vi "Analog_Read_Ex.vi"() -> ()   [LabVIEW 2026]
panel:
  in  "VISA resource name":refnum<visa-resource-name>
  in  "Stop Button":bool
  in  "Canal Read":u8
  out "Waveform Chart":i32(graph)
  out "error out":errorcluster
  # "Ejemplo: Analog Read"
  # "Descripción: Lee un pin analógico del microcontrolador y muestra el valor en un indicador."
  # "Configuracion"
  # "Indicadores"
  # "Control"
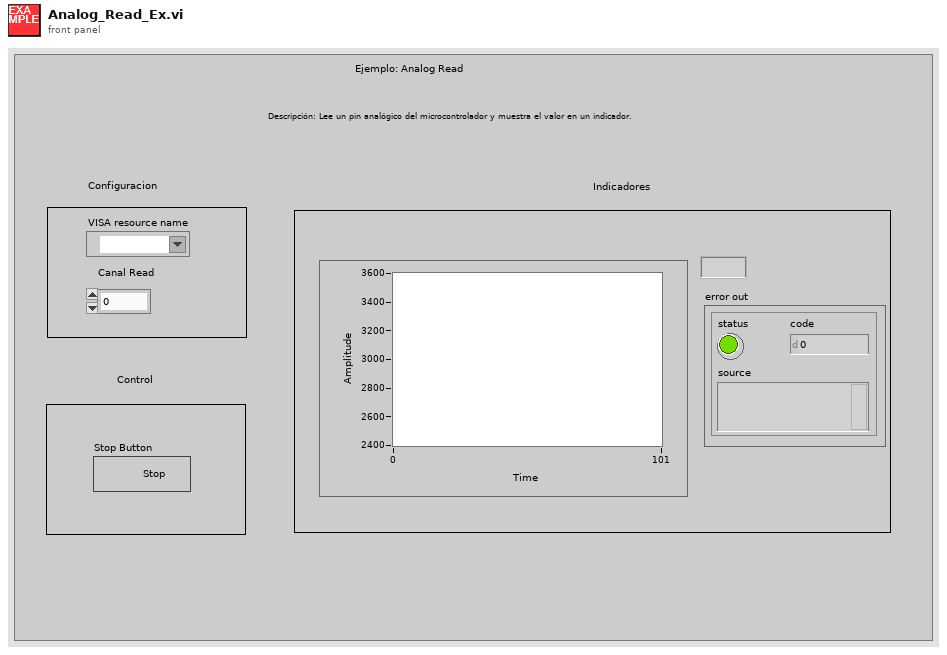
[diagram p1: front panel]
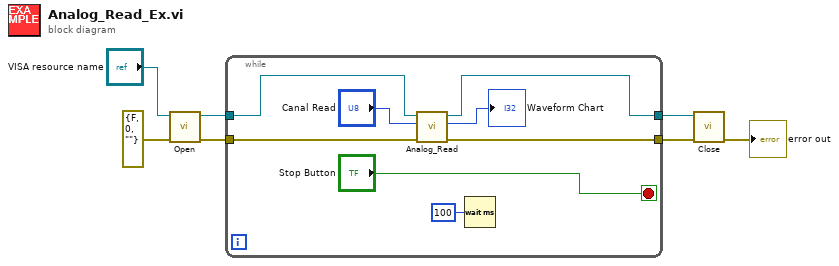
[diagram p0: block diagram]
diagram:
  n1 = call "Open.vi"("error in (no error)"=errorcluster {"status"=FALSE, "code"=0, "source"=""}, "VISA resource name"="VISA resource name") -> ("error out"=w7:errorcluster, "VISA resource name out"=w6:refnum<visa-resource-name>)  [unwired: 8 in]
  n2 = while {
    tunnel: w6 -> [w14]
    tunnel: w7 -> [w13]
    tunnel: [w10] -> w2
    tunnel: [w9] -> w1
    stop <- "Stop Button" stop-if-true
    n3 = call "Analog_Read.vi"("error in (no error)"=w13, "Canal"="Canal Read", "VISA resource name"=w14) -> ("error out"=w9:errorcluster, "Out"=→"Waveform Chart":i32, "VISA resource name out"=w10:refnum<visa-resource-name>)  [unwired: 6 in]
    n4 = Wait (ms)(milliseconds to wait=u32 100) -> ()  [unwired: 1 out]
  }
  n5 = call "Close.vi"("error in (no error)"=w1, "VISA resource name"=w2) -> ("error out"=→"error out":errorcluster)  [unwired: 9 in]
